vi "LabviewOscilloscopeChecksum.vi"(2 "DATA PACKET":string, 3 "ChkSumType":enum16{"ZERO16", "LRC8", "CRC16-CCITT"}(ring)) -> (0 "ChkSum":string, 1 "Checked":bool)   [LabVIEW 2014]
panel:
  # "LabviewOscilloscopeChecksum"
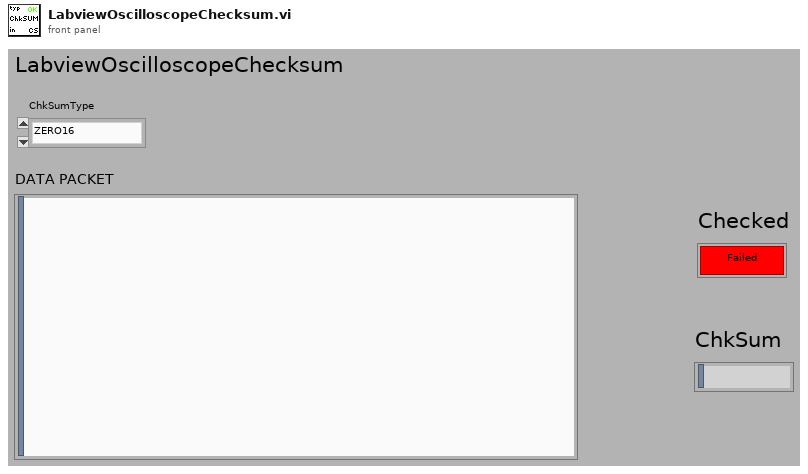
[diagram p1: front panel]
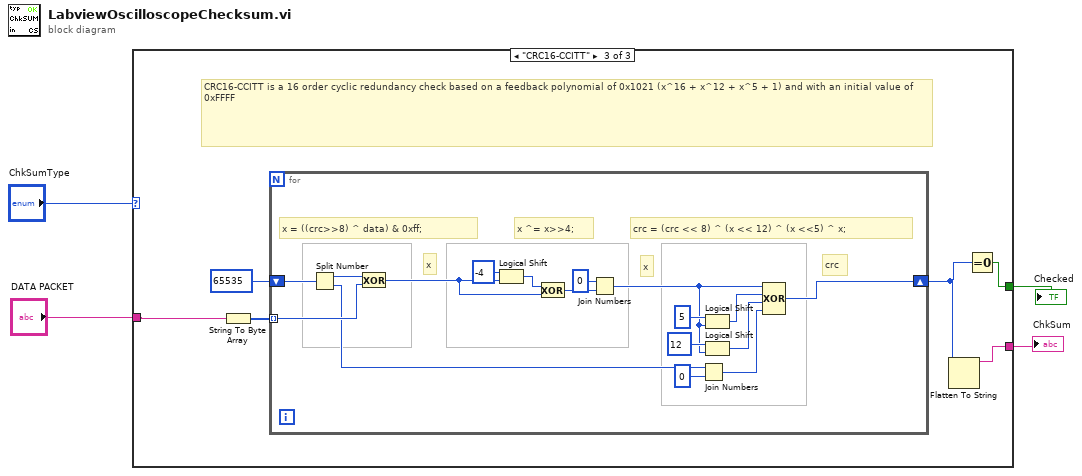
[diagram p0: block diagram]
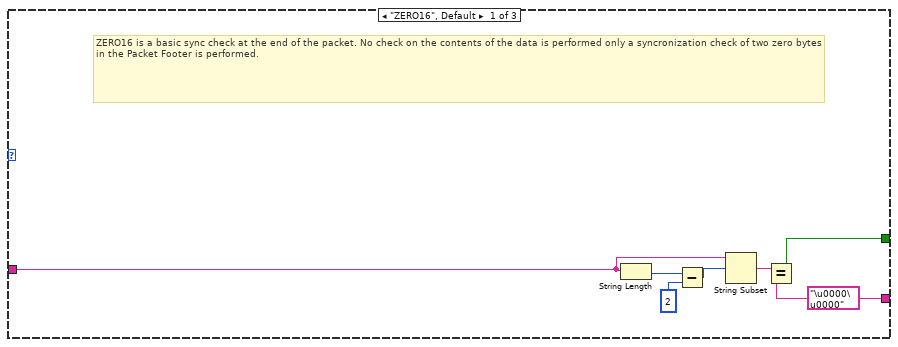
[diagram p2: hidden frame]
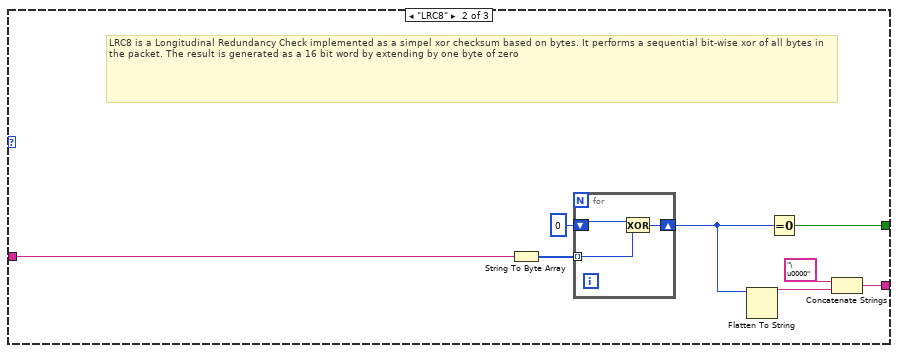
[diagram p3: hidden frame]
diagram:
  n1 = case shown="\"CRC16-CCITT\"" "ChkSumType" {
    tunnel: "DATA PACKET" -> [w11 w19 w26]
    tunnel: [w7 w16 w25] -> w2
    tunnel: [w6 w14 w24] -> w1
    frame "ZERO16", Default {
      w7 = "\u0000\u0000"
      # "ZERO16 is a basic sync check at the end of the packet. No check on the contents of the data is performed only a syncronization check of two zero bytes in the Packet Footer is performed."
      n2 = String Length(string=w11) -> (length=w10:i32)
      n3 = Subtract(x=w10, y=2) -> (x-y=w5:i32)
      n4 = String Subset(string=w11, offset (0)=w5) -> (substring=w8:string)  [unwired: 1 in]
      n5 = Equal?(x=w8, y=w7) -> (x = y?=w6:bool)
    }
    frame "LRC8" {
      # "LRC8 is a Longitudinal Redundancy Check implemented as a simpel xor checksum based on bytes. It performs a sequential bit-wise xor of all bytes in the packet. The result is generated as a 16 bit word by extending by one byte of zero"
      n6 = String To Byte Array(string=w19) -> (unsigned byte array=w18:u8[])
      n7 = for {
        tunnel: w18 -> [w22] mode=indexing
        shift-right: [w20] -> w15
        shift-left: u8 0 -> [w21]
        n8 = Exclusive Or(1:w22, 2:w21) -> (0:w20:u8)
      }
      n9 = Flatten To String(anything=w15) -> (data string=w13:string)  [unwired: 3 in, 2 out]
      n10 = Equal To 0?(x=w15) -> (x = 0?=w14:bool)
      n11 = Concatenate Strings("\u0000", w13) -> (w16:string)
    }
    frame "CRC16-CCITT" {
      # "CRC16-CCITT is a 16 order cyclic redundancy check based on a feedback polynomial of 0x1021 (x^16 + x^12 + x^5 + 1) and with an initial value of 0xFFFF"
      n12 = String To Byte Array(string=w26) -> (unsigned byte array=w28:u8[])
      n13 = for {
        tunnel: w28 -> [w39] mode=indexing
        shift-right: [w29] -> w23
        shift-left: u16 65535 -> [w38]
        # "crc"
        # "crc = (crc << 8) ^ (x << 12) ^ (x <<5) ^ x;"
        # "x"
        # "x ^= x>>4;"
        # "x"
        # "x = ((crc>>8) ^ data) & 0xff;"
        n14 = Split Number(x=w38) -> (hi(x)=w45:u8, lo(x)=w32:u8)
        n15 = Exclusive Or(1:w39, 2:w45) -> (0:w42:u8)
        n16 = Logical Shift(y=i8 -4, x=w42) -> (x << y=w43:u8)
        n17 = Exclusive Or(1:w42, 2:w43) -> (0:w41:u8)
        n18 = Join Numbers(hi=u8 0, lo=w41) -> ((hi.lo)=w34:u16)
        n19 = Join Numbers(hi=w32, lo=u8 0) -> ((hi.lo)=w30:u16)
        n20 = Logical Shift(y=i8 5, x=w34) -> (x << y=w36:u16)
        n21 = Logical Shift(y=i8 12, x=w34) -> (x << y=w33:u16)
        n22 = Compound Arithmetic op=XOR(w34, w36, w33, w30) -> (w29:u16)
      }
      n23 = Flatten To String(anything=w23) -> (data string=w25:string)  [unwired: 3 in, 2 out]
      n24 = Equal To 0?(x=w23) -> (x = 0?=w24:bool)
    }
  }
  "ChkSum" <- w2
  "Checked" <- w1
